vi "06b-arrays.vi"() -> ()   [LabVIEW 2018, in "LV2Julia_examples.lvlib"]
uses:
  LV2Julia_examples.lvlib
  LV2Julia_core/VIs/Server or client state.ctl
  LV2Julia_core/VIs/detailed error info.ctl
  LV2Julia_core/VIs/StackFrame.ctl
  LV2Julia_core/VIs/Commands.ctl
  LV2Julia_core/VIs/ZMQ timeouts.ctl
  0d29fc62-3d1d-4713-a954-9c9e873b3633.vi
  aea790a6-a42b-4eb0-905f-734239196901.vi
  72a46192-383e-4ee5-9465-71670922b82a.vi
  ef5408d4-6538-41d1-b296-fda05a71e4b0.vi
  0fd87d3a-0dd9-45f4-8982-e9f3392e480d.vi
  e4efb182-1b04-4d49-96a3-1defebd055ea.vi
  <vilib>/Analysis/7linalg.llb/Solve Linear Equations (single right hand).vi
  0d29fc62-3d1d-4713-a954-9c9e873b3633.vi/8ee49078-a04b-40cf-aceb-de90d52f19ef.vi
  aea790a6-a42b-4eb0-905f-734239196901.vi/353007a7-a356-474a-8eac-0d4386ef6058.vi
  72a46192-383e-4ee5-9465-71670922b82a.vi/9a7c4f2d-e675-409a-a96a-40bfd606c5f9.vi
  ef5408d4-6538-41d1-b296-fda05a71e4b0.vi/e21b7206-574b-4739-a23f-f6b03aa2b5a4.vi
  0fd87d3a-0dd9-45f4-8982-e9f3392e480d.vi/a484dc78-a8fd-4f8e-92fc-2b44b694d99a.vi
  e4efb182-1b04-4d49-96a3-1defebd055ea.vi/956f82d9-9bd2-463f-b1ac-4d550babe894.vi
  e4efb182-1b04-4d49-96a3-1defebd055ea.vi/96646585-0dd8-4663-891e-f628f50dc7a0.vi
  e4efb182-1b04-4d49-96a3-1defebd055ea.vi/67eea04c-9d13-4b40-9799-894c97b0aeb5.vi
  e4efb182-1b04-4d49-96a3-1defebd055ea.vi/c3cae68e-f011-43a1-90c7-511932c9119b.vi
  <vilib>/Analysis/baseanly.llb/Solve Linear Equations By Cholesky.vi
  <vilib>/Analysis/baseanly.llb/Real Matrix to Compact Array.vi
  <vilib>/Analysis/baseanly.llb/Real Compact Tri-Matrix Linear Eqs.vi
  72a46192-383e-4ee5-9465-71670922b82a.vi/9a7c4f2d-e675-409a-a96a-40bfd606c5f9.vi/d17c7089-7ee8-4662-a957-c6084f5f0cbc.vi
  ef5408d4-6538-41d1-b296-fda05a71e4b0.vi/e21b7206-574b-4739-a23f-f6b03aa2b5a4.vi/2ce2c507-7ab2-4256-a350-c07e3e98c58d.vi
  0fd87d3a-0dd9-45f4-8982-e9f3392e480d.vi/a484dc78-a8fd-4f8e-92fc-2b44b694d99a.vi/0f7293bb-952b-4d9e-a81c-012cedfed96a.vi
  0fd87d3a-0dd9-45f4-8982-e9f3392e480d.vi/a484dc78-a8fd-4f8e-92fc-2b44b694d99a.vi/a01afd5b-5fbd-480c-82a6-7de13792fb26.vi
  0fd87d3a-0dd9-45f4-8982-e9f3392e480d.vi/a484dc78-a8fd-4f8e-92fc-2b44b694d99a.vi/452df562-0e55-46a5-9da0-9746ec63ac9c.vi
  e4efb182-1b04-4d49-96a3-1defebd055ea.vi/956f82d9-9bd2-463f-b1ac-4d550babe894.vi/11ad4541-7f1a-43f7-990d-8cad737a9520.vi
  e4efb182-1b04-4d49-96a3-1defebd055ea.vi/956f82d9-9bd2-463f-b1ac-4d550babe894.vi/1e3e15f7-7400-4596-981c-a908953595fc.vi
  72a46192-383e-4ee5-9465-71670922b82a.vi/9a7c4f2d-e675-409a-a96a-40bfd606c5f9.vi/d17c7089-7ee8-4662-a957-c6084f5f0cbc.vi/0d6d414e-c221-46eb-b9ae-c254e79bf76f.vi
  ef5408d4-6538-41d1-b296-fda05a71e4b0.vi/e21b7206-574b-4739-a23f-f6b03aa2b5a4.vi/2ce2c507-7ab2-4256-a350-c07e3e98c58d.vi/4cac828b-235d-477f-9bd2-cb69159413ed.vi
  e4efb182-1b04-4d49-96a3-1defebd055ea.vi/956f82d9-9bd2-463f-b1ac-4d550babe894.vi/11ad4541-7f1a-43f7-990d-8cad737a9520.vi/f3369d6e-dad0-4ef6-bda0-1534822d836e.vi
  LV2Julia_core/VIs/jl-scripts path.vi
  LV2Julia_core/VIs/check ID validity.vi
  LV2Julia_core/VIs/bindata_descr to JSON.vi
  LV2Julia_core/VIs/check cluster field names.vi
  LV2Julia_core/VIs/concat JSON.vi
  LV2Julia_core/VIs/build request.vi
  LV2Julia_core/VIs/Parse server response.vi
  LV2Julia_core/VIs/log jl exceptions.vi
  <vilib>/Utility/error.llb/Error Cluster From Error Code.vi
  <vilib>/Analysis/7linalg.llb/Solve Linear Eqs (General).vi
  <vilib>/Analysis/7linalg.llb/Solve Linear Eqs (Gen, single right hand).vi
  LV2Julia_core/LV2Julia_core.lvlib
  <vilib>/Analysis/NI_AALPro.lvlib
panel:
  out "LV computation time":dbl
  in  "compare with LV computation":bool=TRUE
  out "Julia call duration (ms)":dbl format="%#.3f"
  out "max difference LV-Jl":dbl format="%#_3e"
  in  "arr size N":u16=4
  out "Solution Vector":dbl[](array[numeric]) format="%.2f"
  out "Known Vector":dbl[](array[numeric])=[22.0, 14.0, 18.0]
  out "Input Matrix (NxN)":dbl[][](array[numeric])=[[1.0, 0.0, 5.0], [4.0, 2.0, 1.0], [2.0, 2.0, 3.0]]
  in  "next":bool
  out "detailed error info":T1
  out "current error":errorcluster
  out "final error":errorcluster
  out "short err code":u8
  in  "stop":bool
  out "ZMQ timeout":bool
  out "Julia script file path":path
  out "temporary script path":path
  out "Jl Server state":T3
  # "Solving a system of linear equations. Optionally comparing Julia and LabVIEW solution.\n\nOn this computer at size N=700 Julia and LV break even at approx. 0.1 s, and for larger arrays Julia call outperforms LV build-in function."
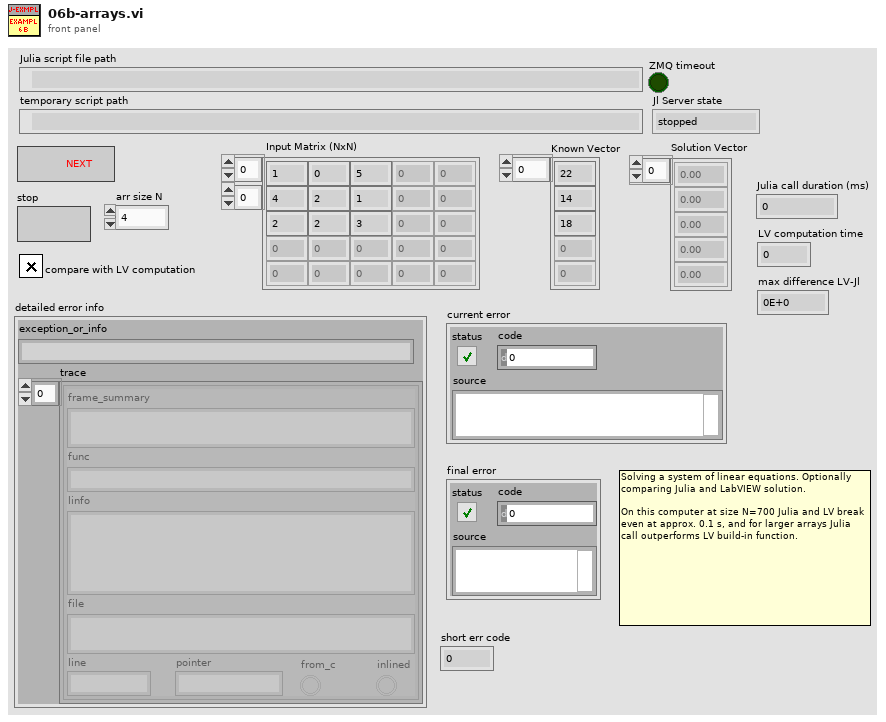
[diagram p1: front panel]
types:
  T1 = typedef "LV2Julia_core.lvlib/detailed error info.ctl" = cluster{"exception_or_info":string, "trace":T2[]}
  T2 = typedef "LV2Julia_core.lvlib/StackFrame.ctl" = cluster{"frame_summary":string, "func":string, "linfo":string, "file":string, "line":i32, "pointer":u64, "from_c":bool, "inlined":bool}
  T3 = typedef "LV2Julia_core.lvlib/Server or client state.ctl" = enum16{"stopped", "running", "unknown"}
  T4 = typedef "LV2Julia_core.lvlib/ZMQ timeouts.ctl" = cluster{"SNDTIMEO":i32, "RCVTIMEO":i32}
  T5 = typedef "LV2Julia_core.lvlib/Commands.ctl" = enum16{"Start Jl-server & Init LV-client", "Send request & Get response ", "Stop Jl-server & Cleanup LV-client", "Cleanup LV-client", "Start Jl-server", "Stop Jl-server", "Init LV-Client", "Cleanup LV-Client", "(not allowed)", "Set LV Client state", "Set Jl Server state", "set ZMQ timeout", "read ZMQ timeout", "read-out state"}
  T6 = typedef "LV2Julia_core.lvlib/Bindata&description.ctl" = cluster{"bindata_descr":T7[], "bindata":u8[]}
  T7 = typedef "LV2Julia_core.lvlib/Bindata description.ctl" = cluster{"nofbytes":i32, "numtype":string, "start":i32, "arrdims":i32[], "kwarg_name":string, "category":string}
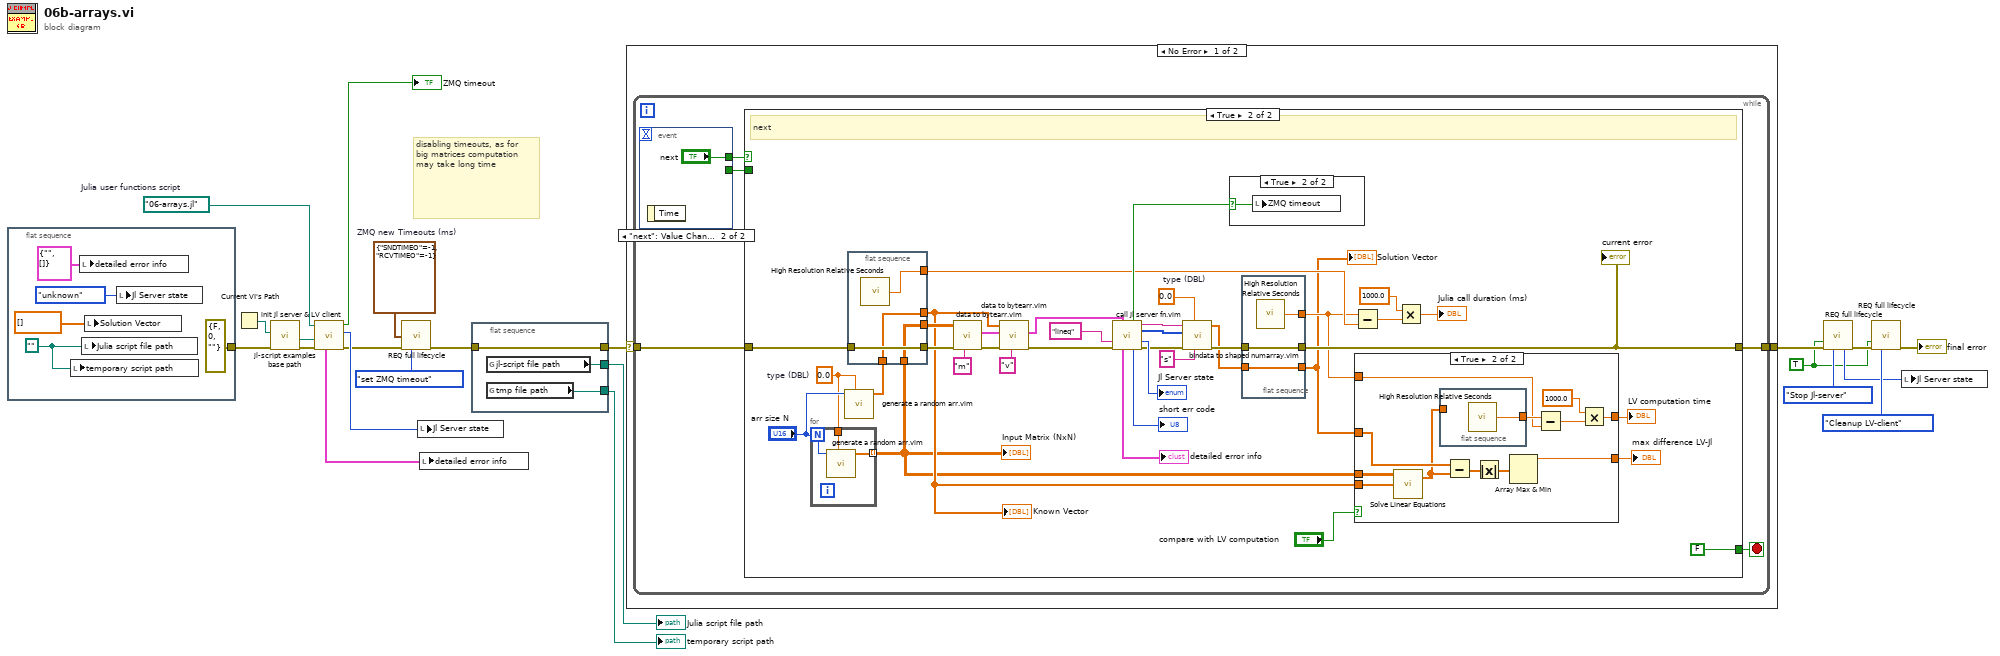
[diagram p0: block diagram]
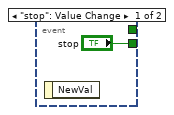
[diagram p2: hidden frame]
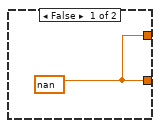
[diagram p4: hidden frame]
diagram:
  w11 = T4 {"SNDTIMEO"=-1, "RCVTIMEO"=-1}  # ZMQ new Timeouts (ms)
  w9 = path "06-arrays.jl"  # Julia user functions script
  w13 = TRUE ("Force command")
  # "disabling timeouts, as for big matrices computation may take long time"
  n1 = flat-sequence {
    tunnel: [errorcluster {"status"=FALSE, "code"=0, "source"=""} ("error in (no error)")] -> w3
    frame #0 {
      w23 = path ""
      n2 = local write "temporary script path"(w23) -> ()
      n3 = local write "detailed error info"(T1 {"exception_or_info"="", "trace"=[]} ("detailed error info")) -> ()
      n4 = local write "Julia script file path"(w23) -> ()
      n5 = local write "Solution Vector"(dbl[] [] ("Server response")) -> ()
      n6 = local write "Jl Server state"(Server_or_client_state."unknown" ("Jl Server state out")) -> ()
    }
  }
  n7 = Current VI's Path() -> (path=w5:path)
  n8 = call "jl-script examples base path.vi"("error in (no error)"=w3, "calling example VI path"=w5) -> ("error out"=w4:errorcluster, "jl-script-examples base path"=w2:path)  [unwired: 8 in]
  n9 = call "init Jl server & LV client.vi"("error in (no error)"=w4, "Base path (not a path)"=w2, "Julia user functions script"=w9) -> ("error out"=w6:errorcluster, "Jl Server state out"=w7:T3, "timeout?"=→"ZMQ timeout":bool, "detailed error info"=w1:T1)  [unwired: 3 in, 2 out]
  n10 = call "REQ full lifecycle.vi"("ZMQ new Timeouts in"=w11, "error in"=w6, "command"=Commands."set ZMQ timeout") -> ("error out"=w10:errorcluster)  [unwired: 6 in, 6 out]
  n11 = local write "Jl Server state"(w7) -> ()
  n12 = local write "detailed error info"(w1) -> ()
  n13 = flat-sequence {
    tunnel: [w30] -> w17
    tunnel: w10 -> [w30]
    tunnel: [w29] -> w15
    tunnel: [w28] -> w16
    frame #0 {
      n14 = global read "jl-scripts path.vi" "jl-script file path"() -> (w29:path)
      n15 = global read "jl-scripts path.vi" "tmp file path"() -> (w28:path)
    }
  }
  n16 = case shown="No Error" w17 {
    selector: w17 -> [w31 w104]
    tunnel: [w32 w104] -> w22
    frame No Error {
      n17 = while {
        tunnel: w31 -> [w36]
        tunnel: [w37] -> w32
        stop <- w34 stop-if-true
        n18 = event shown="[1] \"next\": Value Change" {
          selector: _ -> [_ _]
          dyn-events: _ -> [_ _]
          timeout: _ -> [_ _]
          tunnel: [_ "next"] -> w35
          tunnel: ["stop" _] -> w33
          event "stop": Value Change {
            n19 = event-data() -> ()  [unwired: 1 in, 1 out]
          }
          event "next": Value Change {
            n20 = event-data() -> ()  [unwired: 1 in, 1 out]
          }
        }
        n21 = case shown="True" w35 {
          tunnel: [w41 w53] -> w37
          tunnel: w36 -> [w41 w58]
          tunnel: [w40 FALSE ("stop this VI only")] -> w34
          tunnel: w33 -> [w40 _]
          frame False {
            # "stop"
          }
          frame True {
            w70 = 0.0  # type (DBL)
            w73 = 0.0  # type (DBL)
            # "next"
            n22 = for {
              N: "arr size N" -> [w100]
              tunnel: [w102] -> w46 mode=indexing
              tunnel: w70 -> [w101]
              n23 = call "generate a random arr.vim"("type in"=w101, "arr size"=w100) -> ("float out"=w102:dbl[])  [unwired: 5 in, 4 out]
            }
            "Input Matrix (NxN)" <- w46
            n24 = call "generate a random arr.vim"("type in"=w70, "arr size"="arr size N") -> ("float out"=w55:dbl[])  [unwired: 5 in, 4 out]
            n25 = flat-sequence {
              tunnel: [w99] -> w57
              tunnel: w58 -> [w99]
              tunnel: w46 -> [w98]
              tunnel: [w98] -> w56
              tunnel: [w97] -> w47
              tunnel: w55 -> [w97]
              tunnel: [w96] -> w52
              frame #0 {
                n26 = call <vilib>:"High Resolution Relative Seconds.vi"() -> ("relative seconds"=w96:dbl)
              }
            }
            n27 = call "data to bytearr.vim"("kwarg_name"="m", "error in (no error)"=w57, "data in"=w56) -> ("error out"=w77:errorcluster, "Bindata & descr out"=w76:T6)  [unwired: 6 in, 1 out]
            n28 = call "data to bytearr.vim"("kwarg_name"="v", "error in (no error)"=w77, "Bindata & descr in"=w76, "data in"=w47) -> ("error out"=w59:errorcluster, "Bindata & descr out"=w63:T6)  [unwired: 5 in, 1 out]
            n29 = call "call Jl server fn.vim"("Bindata & descr in"=w63, "fun2call"="lineq" ("Julia function name"), "error in (no error)"=w59) -> ("timeout?"=w62:bool, "JSON received"=w61:string, "binary data received"=w60:u8[], "Jl Server state out"=→"Jl Server state":T3, "detailed error info"=→"detailed error info":T1, "return code"=→"short err code":u8, "error out"=w64:errorcluster)  [unwired: 6 in]
            n30 = call "bindata to shaped numarray.vim"("name"="s" ("kwarg_name"), "element type"=w73, "error in (no error)"=w64, "binary data"=w60, "JSON in"=w61) -> ("error out"=w54:errorcluster, "numarray 1D"=w43:dbl[])  [unwired: 1 in, 4 out]
            n31 = case shown="True" w62 {
              selector: w62 -> [_ w103]
              frame False {
              }
              frame True {
                n32 = local write "ZMQ timeout"(w103) -> ()
              }
            }
            n33 = flat-sequence {
              tunnel: [w95] -> w53
              tunnel: w54 -> [w95]
              tunnel: [w94] -> w45
              tunnel: [w93] -> w42
              tunnel: w43 -> [w93]
              frame #0 {
                n34 = call <vilib>:"High Resolution Relative Seconds.vi"() -> ("relative seconds"=w94:dbl)
              }
            }
            n35 = Subtract(x=w45, y=w52) -> (x-y=w50:dbl)
            n36 = case shown="True" "compare with LV computation" {
              tunnel: w42 -> [_ w91]
              tunnel: [w79 w88] -> w69
              tunnel: w46 -> [_ w87]
              tunnel: w47 -> [_ w86]
              tunnel: w45 -> [_ w81]
              tunnel: [w79 w80] -> w44
              frame False {
                w79 = nan
              }
              frame True {
                n37 = call-poly <vilib>:"Solve Linear Equations.vi"("Known Vector"=w86, "Input Matrix"=w87) -> ("Solution Vector"=w85:dbl[])  [unwired: 1 in, 1 out]
                n38 = flat-sequence {
                  tunnel: w85 -> [_]
                  tunnel: [w92] -> w82
                  frame #0 {
                    n39 = call <vilib>:"High Resolution Relative Seconds.vi"() -> ("relative seconds"=w92:dbl)
                  }
                }
                n40 = Subtract(x=w91, y=w85) -> (x-y=w90:dbl[])
                n41 = Absolute Value(x=w90) -> (abs(x)=w89:dbl[])
                n42 = Array Max & Min(array=w89) -> (max value=w88:dbl)  [unwired: 3 out]
                n43 = Subtract(x=w82, y=w81) -> (x-y=w83:dbl)
                n44 = Multiply(x=1000.0, y=w83) -> (x*y=w80:dbl)
              }
            }
            "max difference LV-Jl" <- w69
            "LV computation time" <- w44
            n45 = Multiply(x=1000.0, y=w50) -> (x*y=→"Julia call duration (ms)":dbl)
            "current error" <- w53
            "Known Vector" <- w47
            "Solution Vector" <- w42
          }
        }
      }
    }
    frame Error {
    }
  }
  n46 = call "REQ full lifecycle.vi"("Force command"=w13, "error in"=w22, "command"=Commands."Stop Jl-server") -> ("Jl Server state out"=w14:T3, "error out"=w20:errorcluster)  [unwired: 6 in, 5 out]
  n47 = call "REQ full lifecycle.vi"("Force command"=w13, "error in"=w20, "command"=Commands."Cleanup LV-client") -> ("error out"=→"final error":errorcluster)  [unwired: 6 in, 6 out]
  n48 = local write "Jl Server state"(w14) -> ()
  "temporary script path" <- w16
  "Julia script file path" <- w15
